vi "Save Entry.vi"(7 "Time Entry Store in":refnum<class "Time Entry Store-INI.lvclass">, 8 "error in (no error)":errorcluster, 10 "Project Store":refnum<class "Project Store.lvclass">, 11 "Time Entry":T1) -> (0 "error out":errorcluster, 5 "Time Entry Store out":refnum<class "Time Entry Store-INI.lvclass">)   [LabVIEW 2024, in "Time Entry Store-INI.lvclass"]
doc: "Saves a time entry into the month file chosen by its Start Time in UTC (YYYY-MM.ini) - creating the file, adding the row, or overwriting the row with the same ID. The file is rewritten with the [_Meta] section and every row sorted by Start Time. Project Store is optional: when wired its Get Project by ID and Get Task by ID supply the Project Name and Task Name labels, otherwise they are written empty. If an entry is moved to another month by changing its Start Time, delete it with its OLD Start Time first.\n\nGenerated by: Claude"
uses:
  Time Entry Store-INI.lvclass
  Project Store/Project Store.lvclass
  Rows/Time Entry.ctl
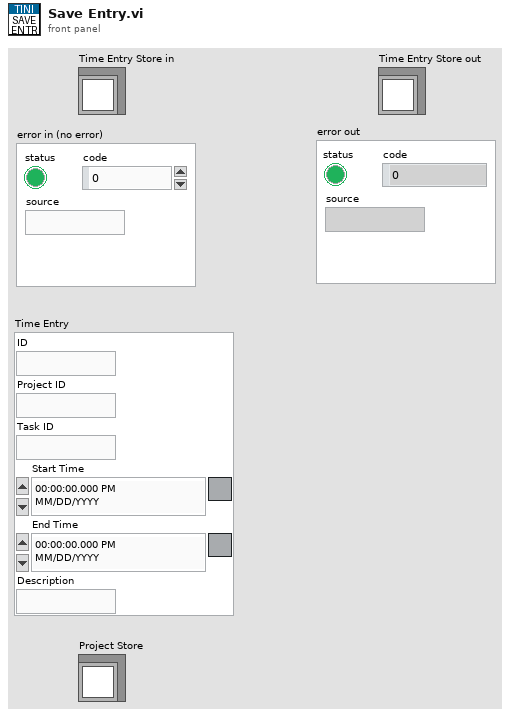
[diagram p1: front panel]
types:
  T1 = typedef "Time Entry.ctl" = cluster{"ID":string, "Project ID":string, "Task ID":string, "Start Time":timestamp, "End Time":timestamp, "Description":string}
  T2 = typedef "Time Entry List.ctl" = T1[]
  T3 = typedef "Project.ctl" = cluster{"ID":string, "Name":string, "Active":bool, "Sort Order":i32}
  T4 = typedef "Task.ctl" = cluster{"ID":string, "Project ID":string, "Name":string, "Active":bool, "Sort Order":i32}
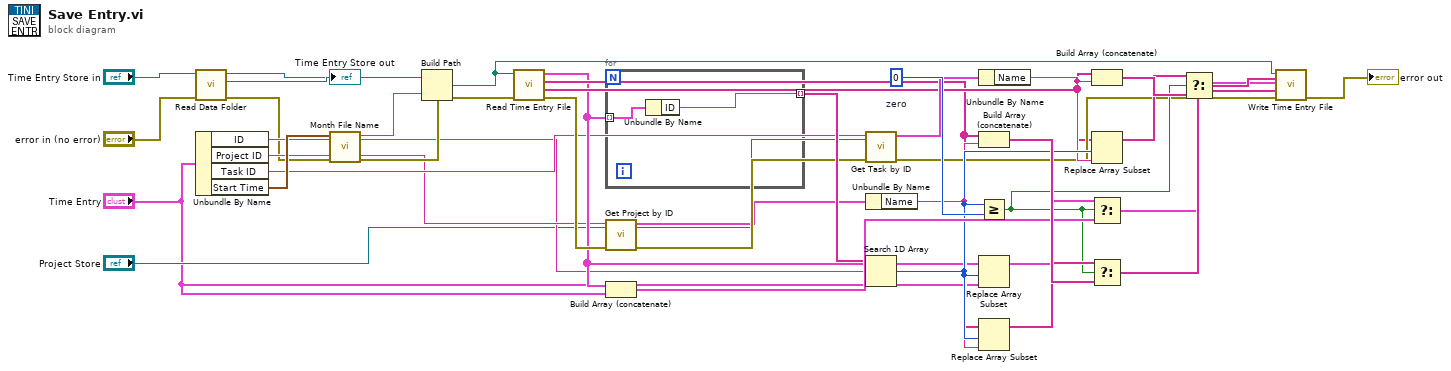
[diagram p0: block diagram]
diagram:
  w28 = 0  # zero
  n1 = call-dynamic "Read Data Folder.vi"("error in (no error)"="error in (no error)", "Time Entry Store-INI in"="Time Entry Store in") -> ("error out"=w5:errorcluster, "Data Folder"=w7:path, "Time Entry Store-INI out"=→"Time Entry Store out":refnum<class "Time Entry Store-INI.lvclass">)  [unwired: 7 in]
  n2 = Unbundle By Name("Time Entry") -> ("ID"=w8:string, "Project ID"=w9:string, "Task ID"=w10:string, "Start Time"=w11:timestamp)
  n3 = call "Month File Name.vi"("error in (no error)"=w5, "Start Time"=w11) -> ("error out"=w13:errorcluster, "File Name"=w12:string)  [unwired: 8 in]
  n4 = Build Path(base path=w7, name or relative path=w12) -> (appended path=w14:path)
  n5 = call "Read Time Entry File.vi"("error in (no error)"=w13, "File Path"=w14) -> ("error out"=w18:errorcluster, "Task Names"=w17:string[], "Project Names"=w16:string[], "Time Entries"=w15:T2)  [unwired: 6 in]
  n6 = for {
    tunnel: w15 -> [w40] mode=indexing
    tunnel: [w41] -> w26 mode=indexing
    n7 = Unbundle By Name(w40) -> ("ID"=w41:string)
  }
  n8 = call-dynamic "Get Project by ID.vi"("Project Store in"="Project Store", "error in (no error)"=w18, "ID"=w9) -> ("error out"=w21:errorcluster, "Project"=w20:T3, "Project Store out"=w19:refnum<class "Project Store.lvclass">)  [unwired: 5 in, 1 out]
  n9 = Build Array (concatenate)(w15, "Time Entry") -> (w33:T2)
  n10 = call-dynamic "Get Task by ID.vi"("Project Store in"=w19, "error in (no error)"=w21, "ID"=w10) -> ("error out"=w23:errorcluster, "Task"=w22:T4)  [unwired: 5 in, 2 out]
  n11 = Unbundle By Name(w20) -> ("Name"=w24:string)
  n12 = Search 1D Array(1D array=w26, element=w8) -> (index of element=w27:i32)  [unwired: 1 in]
  n13 = Unbundle By Name(w22) -> ("Name"=w25:string)
  n14 = Build Array (concatenate)(w16, w24) -> (w34:string[])
  n15 = Greater Or Equal?(x=w27, y=w28) -> (x >= y?=w29:bool)
  n16 = Replace Array Subset(array=w15, new element="Time Entry", index=w27) -> (w30:T2)
  n17 = Replace Array Subset(array=w16, new element=w24, index=w27) -> (w31:string[])
  n18 = Build Array (concatenate)(w17, w25) -> (w35:string[])
  n19 = Replace Array Subset(array=w17, new element=w25, index=w27) -> (w32:string[])
  n20 = Select(t=w30, s=w29, f=w33) -> (s? t:f=w36:T2)
  n21 = Select(t=w31, s=w29, f=w34) -> (s? t:f=w37:string[])
  n22 = Select(t=w32, s=w29, f=w35) -> (s? t:f=w38:string[])
  n23 = call "Write Time Entry File.vi"("Task Names"=w38, "error in (no error)"=w23, "Project Names"=w37, "Time Entries"=w36, "File Path"=w14) -> ("error out"=→"error out":errorcluster)  [unwired: 6 in]
